vi "gps data sorting.vi"(10 "input string":string) -> (1 "unsigned 32bit integer":u32, 2 "Array 5":string[](array[string]))   [LabVIEW 2023]
uses:
  <vilib>/regexp/Match Regular Expression.xnode
panel:
  out "Array 4":string[][](array[string])
  out "string array":string[](array[string])
  out "length":i32
  out "after match":string
  # "273287"
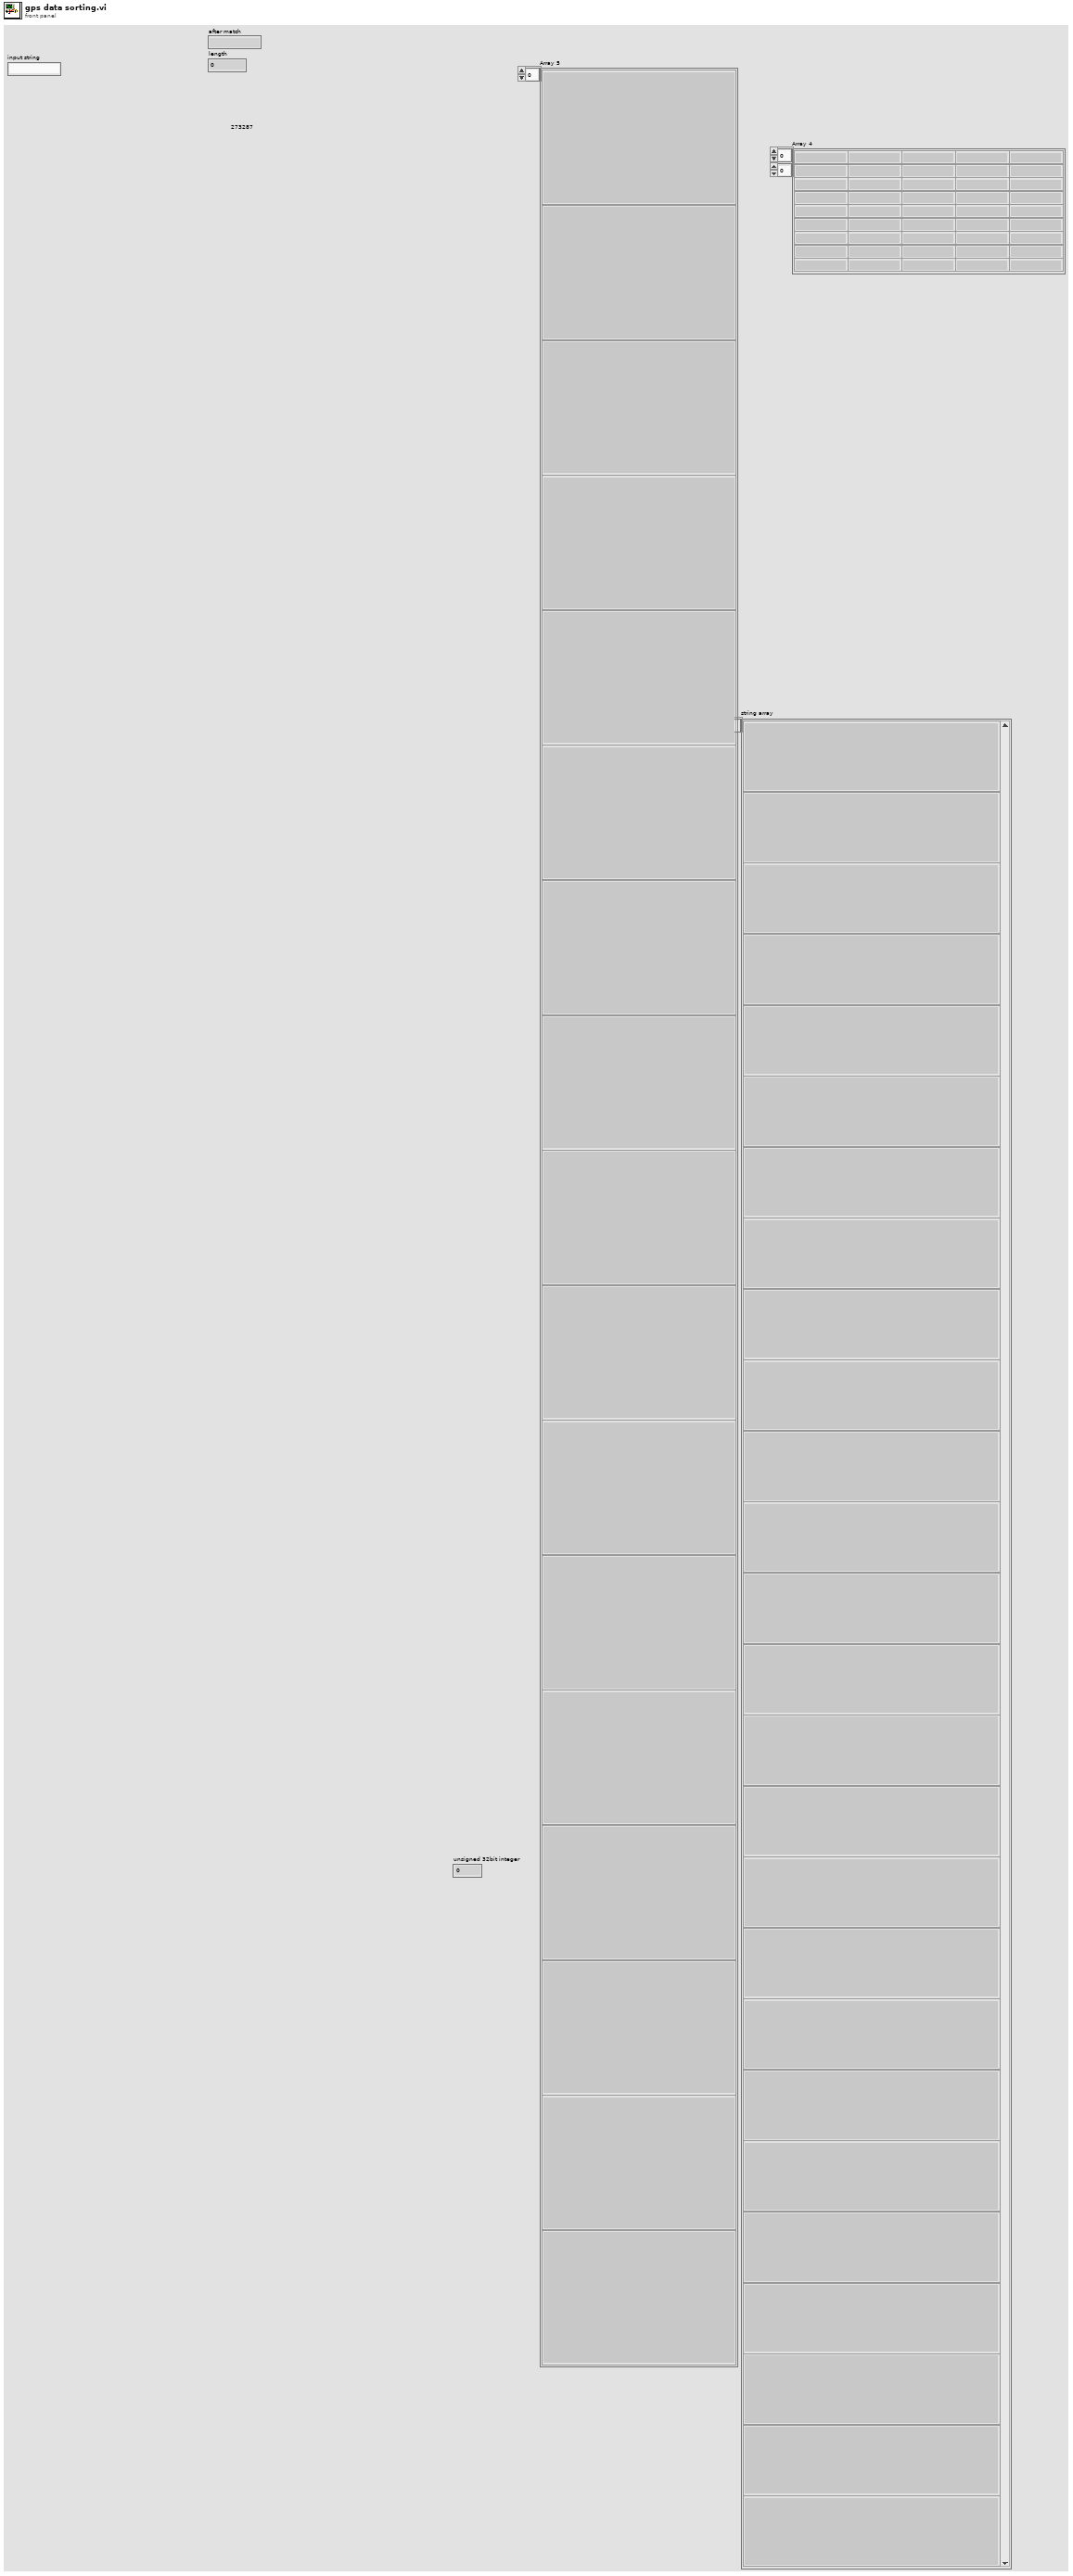
[diagram p1: front panel]
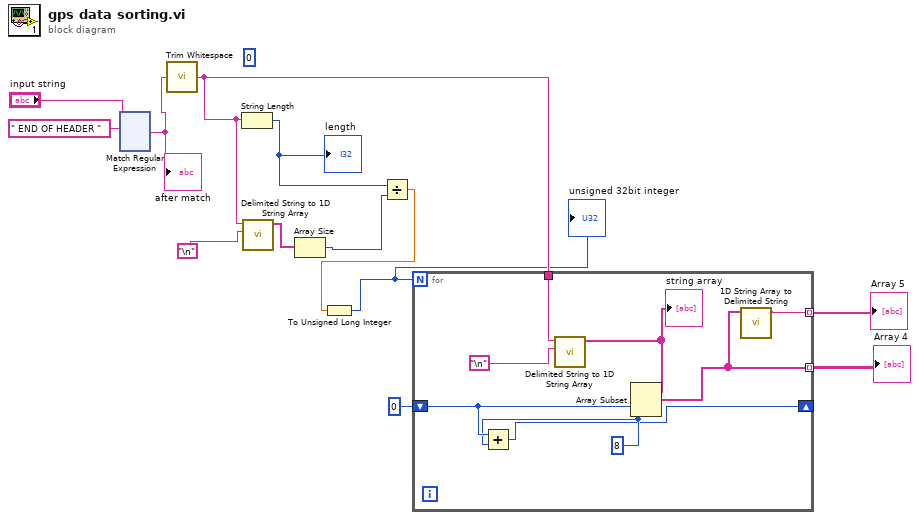
[diagram p0: block diagram]
diagram:
  (unwired) 0 ("Numeric")
  n1 = xnode "Match Regular Expression"("input string"="input string", "regular expression"=" END OF HEADER ") -> ("after match"=w12:string)  [unwired: 4 in, 4 out]
  "after match" <- w12
  n2 = call <vilib>:"Trim Whitespace.vi"("string"=w12) -> ("trimmed string"=w7:string)  [unwired: 1 in]
  n3 = String Length(string=w7) -> (length=w5:i32)
  "length" <- w5
  n4 = call <vilib>:"Delimited String to 1D String Array.vi"("delimiter"="\n", "delimited string"=w7) -> ("string array"=w6:string[])  [unwired: 9 in]
  n5 = Array Size(array=w6) -> (size(s)=w4:i32)
  n6 = Divide(x=w5, y=w4) -> (x/y=w3:dbl)
  n7 = To Unsigned Long Integer(number=w3) -> (unsigned 32bit integer=w1:u32)
  "unsigned 32bit integer" <- w1
  n8 = for {
    N: w1 -> [_]
    tunnel: w7 -> [w21]
    shift-right: [w16] -> _
    shift-left: 0 ("index") -> [w18]
    tunnel: [w15] -> w10 mode=indexing
    tunnel: [w14] -> w9 mode=indexing
    w17 = 8 ("length")
    n9 = Add(x=w18, y=w17) -> (x+y=w16:i32)
    n10 = call <vilib>:"Delimited String to 1D String Array.vi"("delimiter"="\n", "delimited string"=w21) -> ("string array"=w19:string[])  [unwired: 9 in]
    "string array" <- w19
    n11 = Array Subset(array=w19, index=w18, length=w17) -> (w15:string[])
    n12 = call <vilib>:"1D String Array to Delimited String.vi"("string array"=w15) -> ("delimited string"=w14:string)  [unwired: 10 in]
  }
  "Array 4" <- w10
  "Array 5" <- w9
